vi "Read VI and FP Refs.vi"(0 "GUI View in":refnum<class "GUI View.lvclass">, 7 "View Hierarchy Level":i32, 11 "error in (no error)":errorcluster) -> (4 "GUI View out":refnum<class "GUI View.lvclass">, 6 "VI Ref":refnum<vi>, 8 "FP Ref":refnum<vi>, 10 "View Found":bool, 15 "error out":errorcluster)   [LabVIEW 2023, in "GUI Views.lvlib" / "GUI View.lvclass"]
uses:
  GUI View.lvclass
  GUI View.lvclass/GUI View.ctl
  <vilib>/ErrorRing/Error Ring.xnode
  <vilib>/Utility/error.llb/Error Cluster From Error Code.vi
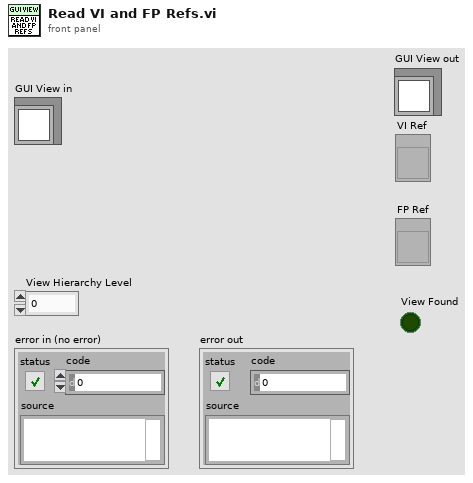
[diagram p1: front panel]
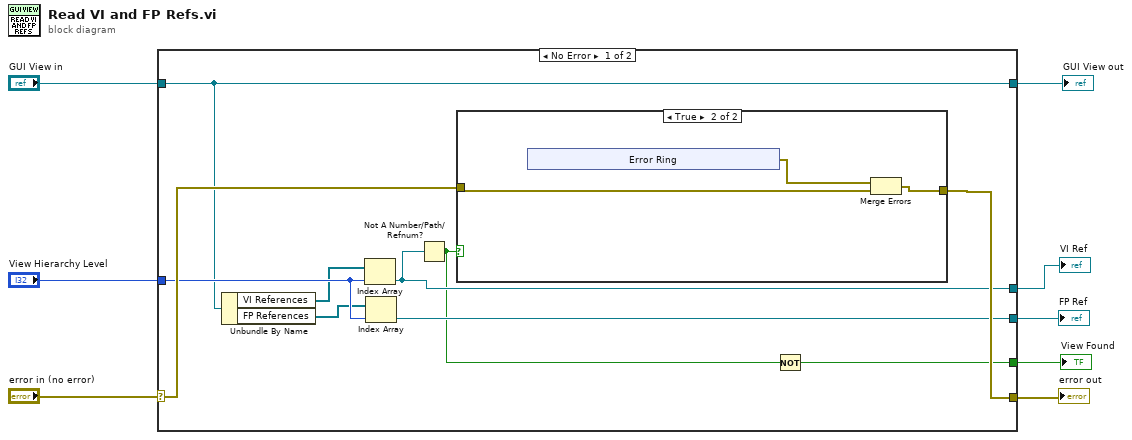
[diagram p0: block diagram]
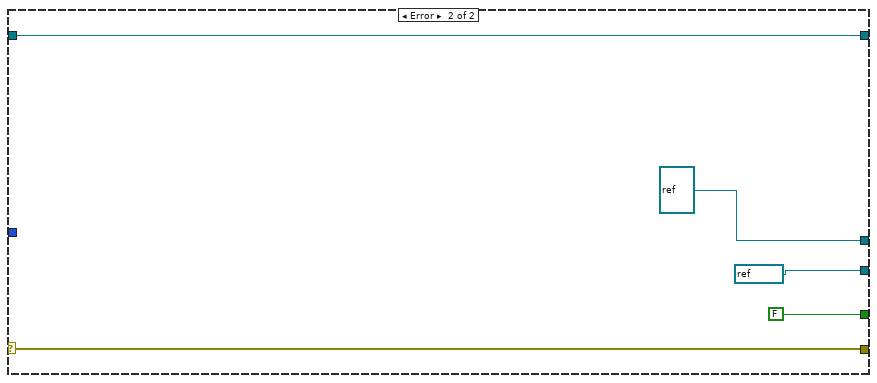
[diagram p3: hidden frame]
diagram:
  n1 = case shown="No Error" "error in (no error)" {
    selector: "error in (no error)" -> [w17 w30]
    tunnel: [w18 w30] -> w8
    tunnel: "GUI View in" -> [w10 w31]
    tunnel: "View Hierarchy Level" -> [w16 _]
    tunnel: [w10 w31] -> w4
    tunnel: [w15 refnum<vi> refnum ("Panel")] -> w3
    tunnel: [w14 refnum<vi> refnum ("reference out")] -> w2
    tunnel: [w9 FALSE] -> w1
    frame No Error {
      n2 = Unbundle By Name(w10) -> ("VI References"=w12:refnum<vi>[], "FP References"=w11:refnum<vi>[])
      n3 = Index Array(array=w12, index=w16) -> (element=w14:refnum<vi>)
      n4 = Index Array(array=w11, index=w16) -> (element=w15:refnum<vi>)
      n5 = Not A Number/Path/Refnum?(number/path/refnum=w14) -> (NaN/Path/Refnum?=w13:bool)
      n6 = case shown="True" w13 {
        tunnel: w17 -> [w19 w21]
        tunnel: [w19 w22] -> w18
        frame False {
        }
        frame True {
          n7 = xnode "Error Ring"() -> ("error out"=w20:errorcluster)
          n8 = Merge Errors(w20, w21) -> (w22:errorcluster)
        }
      }
      n9 = Not(x=w13) -> (.not. x?=w9:bool)
    }
    frame Error {
    }
  }
  "error out" <- w8
  "GUI View out" <- w4
  "FP Ref" <- w3
  "VI Ref" <- w2
  "View Found" <- w1
